vi "Get tag.vi"(8 "error in (no error)":errorcluster, 10 "TagName":string="phygbuTag", 11 "reference":refnum<vi>) -> (0 "error out":errorcluster, 1 "Tag Value":string, 2 "Tag Found ?":bool, 3 "reference Out":refnum<vi>, 5 "Persistant":bool)   [LabVIEW 2012, in "Scripting Tools.lvlib"]
doc: "Returns the string tag set by Set Tag.vi on a LabVIEW object identified by the Reference input."
uses:
  Scripting Tools.lvlib
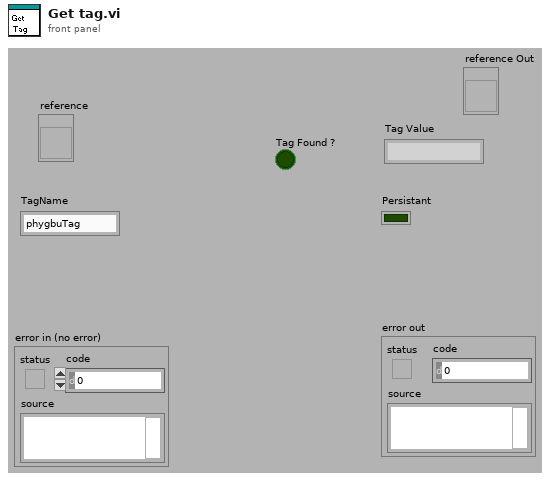
[diagram p1: front panel]
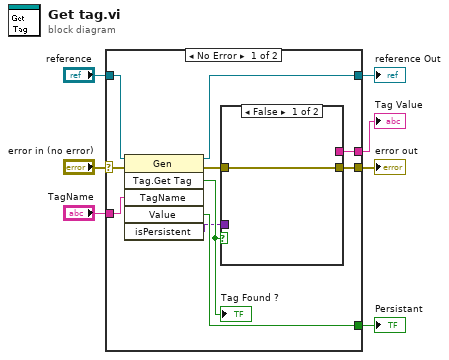
[diagram p0: block diagram]
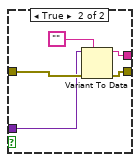
[diagram p2: hidden frame]
diagram:
  n1 = case shown="No Error" "error in (no error)" {
    selector: "error in (no error)" -> [w8 w25]
    tunnel: "reference" -> [w17 w24]
    tunnel: "TagName" -> [w16 _]
    tunnel: [w15 _] -> w5
    tunnel: [w13 _] -> w4
    tunnel: [w10 w25] -> w3
    tunnel: [w9 w24] -> w2
    frame No Error {
      n2 = invoke on="Invoke Node" class="Gen" method="Tag.Get Tag"(reference=w17, error in=w8, "TagName"=w16) -> (reference out=w9:refnum<vi>, error out=w12:errorcluster, "GetTag"=w14:bool, "Value"=w15:bool, "isPersistent"=w11:variant)  [unwired: 3 in, 1 out]
      "Tag Found ?" <- w14
      n3 = case shown="False" w14 {
        tunnel: [_ w23] -> w13
        tunnel: w12 -> [w18 w22]
        tunnel: w11 -> [_ w21]
        tunnel: [w18 w19] -> w10
        frame False {
        }
        frame True {
          n4 = Variant To Data(error in=w22, type="" ("Empty String Constant"), Variant=w21) -> (data=w23:string, error out=w19:errorcluster)
        }
      }
    }
    frame Error {
    }
  }
  "Tag Value" <- w4
  "Persistant" <- w5
  "error out" <- w3
  "reference Out" <- w2
